vi "Delay Miliseconds.vi"(8 "error in (no error)":errorcluster, 11 "ms":u32=1000) -> (0 "error out":errorcluster)   [LabVIEW 2020, in "wiringPi.lvlib"]
doc: "<b>_______________________________________________________________</b>\n** Author: Juan José Villacorta\n** LabVIEW wrapper for C library <b> wiringPi </b>,\n** https://github.com/WiringPi/WiringPi\n<b>_______________________________________________________________</b>\n\n/*\n * delay:\n * Wait for some number of milliseconds\n *********************************************************************************\n */"
uses:
  wiringPi.lvlib
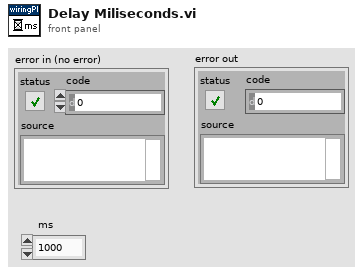
[diagram p1: front panel]
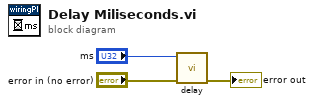
[diagram p0: block diagram]
diagram:
  n1 = call "delay.vi"("error in (no error)"="error in (no error)", "ms"="ms") -> ("error out"=→"error out":errorcluster)  [unwired: 9 in]
